vi "Motion_xyz_circular.vi"(6 "T":dbl, 7 "One_or_negativeone":dbl, 8 "Error IN":errorcluster, 10 "Initial State":dbl[][](array[numeric]), 11 "Constants IN":T2) -> (0 "Error OUT":errorcluster, 2 "Motion Sequence":T1, 3 "Constants OUT":T2)   [LabVIEW 2019]
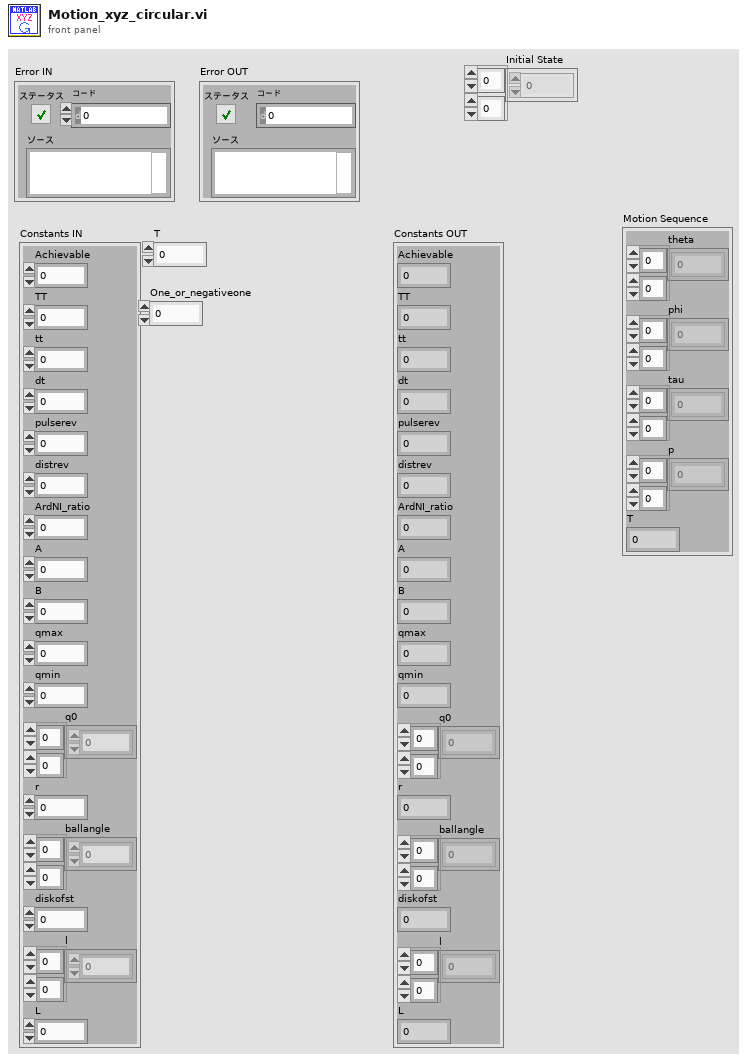
[diagram p1: front panel]
types:
  T1 = cluster{"theta":dbl[][], "phi":dbl[][], "tau":dbl[][], "p":dbl[][], "T":dbl}
  T2 = cluster{"Achievable":dbl, "TT":dbl, "tt":dbl, "dt":dbl, "pulserev":dbl, "distrev":dbl, "ArdNI_ratio":dbl, "A":dbl, "B":dbl, "qmax":dbl, "qmin":dbl, "q0":dbl[][], "r":dbl, "ballangle":dbl[][], "diskofst":dbl, "l":dbl[][], "L":dbl}
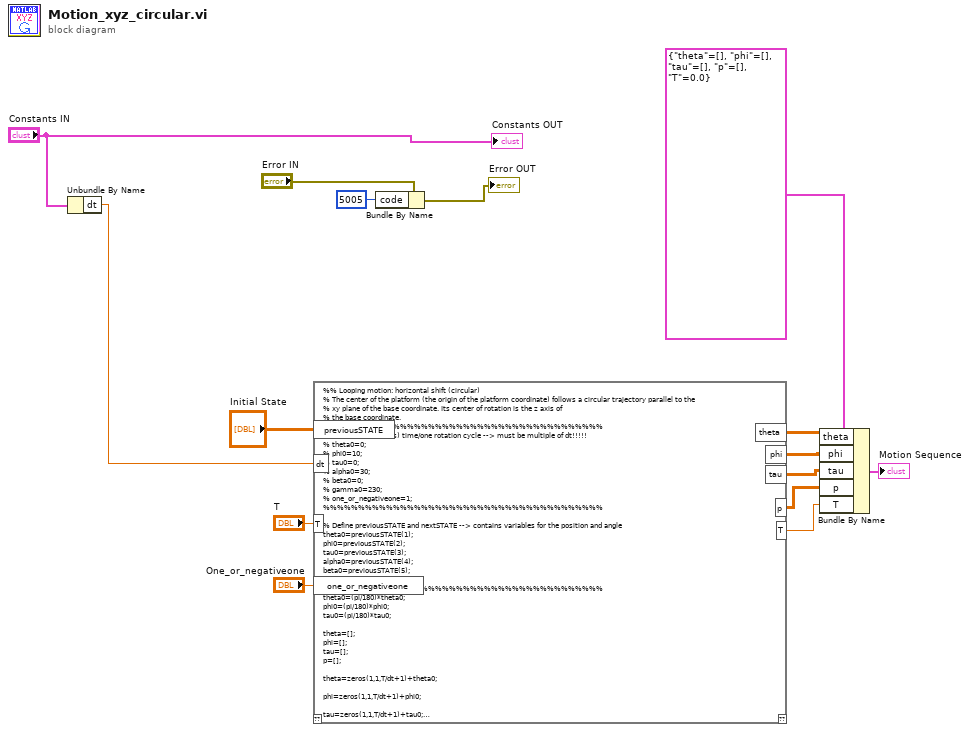
[diagram p0: block diagram]
diagram:
  n1 = Unbundle By Name("Constants IN") -> ("dt"=w1:dbl)
  n2 = script code="%% Looping motion: horizontal shift (circular) \n% The center of the platform (the origin of the platform coordinate) follows a circular trajectory parallel to the\n% xy plane of the base coordinate. Its center of rotation is the z axis of\n% the base coordinate.\n%%%%%%%%%%%%%%%%%%%%%%%%%%%%%%%%%%%%%%%%\n% T=5000;\t\t\t\t\t\t\t% (ms) time/one rotation cycle --> must be multiple of dt!!!!!\n% theta0=0;\n% phi0=10;\n% tau0=0;\n% alpha0=30;\n% beta0=0;\n% gamma0=230;\n% one_or_negativeone=1;\n%%%%%%%%%%%%%%%%%%%%%%%%%%%%%%%%%%%%%%%%\n\n% Define previousSTATE and nextSTATE --> contains variables for the position and angle\ntheta0=previousSTATE(1);\nphi0=previousSTATE(2);\ntau0=previousSTATE(3);\nalpha0=previousSTATE(4);\nbeta0=previousSTATE(5);\ngamma0=previousSTATE(6);\n%%%%%%%%%%%%%%%%%%%%%%%%%%%%%%%%%%%%%%%%\ntheta0=(pi/180)*theta0;\nphi0=(pi/180)*phi0;\ntau0=(pi/180)*tau0;\n\ntheta=[];\nphi=[];\ntau=[];\np=[];\n\ntheta=zeros(1,1,T/dt+1)+theta0;\n\nphi=zeros(1,1,T/dt+1)+phi0;\n\ntau=zeros(1,1,T/dt+1)+tau0;\n\np=zeros(3,T/dt+1,1);\np=cos(one_or_negativeone.*[0:2*pi*dt/T:2*pi]).*[alpha0;beta0;0]+sin(one_or_negativeone.*[0:2*pi*dt/T:2*pi]).*[-beta0;alpha0;0]+[0;0;gamma0];\np=permute(p,[1,3,2]);\np=p+zeros(3,6,T/dt+1);"("previousSTATE"="Initial State", "T"="T", "one_or_negativeone"="One_or_negativeone", "dt"=w1) -> ("theta"=w12:dbl[][], "phi"=w11:dbl[][], "tau"=w10:dbl[][], "p"=w9:dbl[][], "T"=w4:dbl)  [unwired: 1 in, 1 out]
  n3 = Bundle By Name(cluster="Error IN", "code"=5005) -> (→"Error OUT":errorcluster)
  n4 = Bundle By Name(cluster=T1 {"theta"=[], "phi"=[], "tau"=[], "p"=[], "T"=0.0}, "theta"=w12, "phi"=w11, "tau"=w10, "p"=w9, "T"=w4) -> (→"Motion Sequence":T1)
  "Constants OUT" <- "Constants IN"
